vi "Return client handle.vi"(8 "error in (no error)":errorcluster, 9 "headers":T1[](array[typedef]), 10 "http-client":refnum<class "http-client.lvclass">, 11 "REST Client in":refnum<class "REST Client.lvclass">) -> (0 "error out":errorcluster, 3 "REST Client out":refnum<class "REST Client.lvclass">)   [LabVIEW 2020, in "REST Client.lvlib" / "REST Client.lvclass"]
uses:
  REST Client.lvclass
  http-client/http-client.lvclass
  HTTP Header.ctl
  <vilib>/NI/Advanced HTTP Client/Header--Combo Box.ctl
  REST Client.lvclass/REST Client.ctl
  <vilib>/NI/Advanced HTTP Client/Session.lvclass
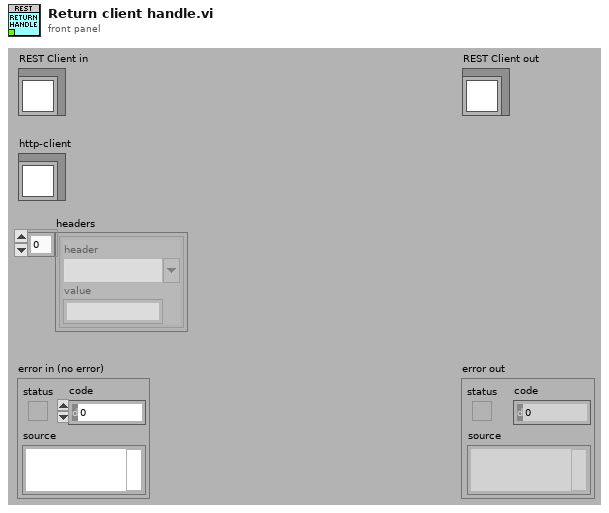
[diagram p1: front panel]
types:
  T1 = typedef "REST Client.lvlib/REST Client.lvclass/HTTP Header.ctl" = cluster{"header":T2, "value":string}
  T2 = typedef "lib_NI_Advanced HTTP Client.lvlib/Session.lvclass/Header--Combo Box.ctl" = string
  T3 = cluster{"http-client":refnum<class "http-client.lvclass">, "headers":T1[]}
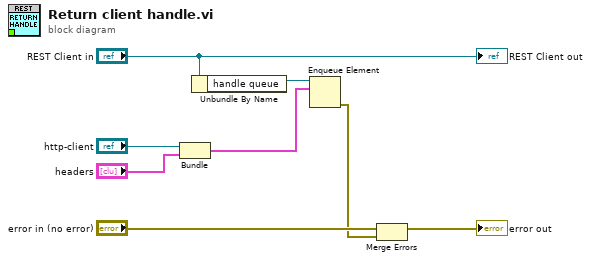
[diagram p0: block diagram]
diagram:
  n1 = Bundle("http-client"="http-client", "headers"="headers") -> (w5:T3)  [unwired: 1 in]
  n2 = Unbundle By Name("REST Client in") -> ("handle queue"=w6:refnum<queue>)
  n3 = Enqueue Element(queue=w6, element=w5) -> (error out=w3:errorcluster)  [unwired: 2 in, 2 out]
  n4 = Merge Errors("error in (no error)", w3) -> (→"error out":errorcluster)
  "REST Client out" <- "REST Client in"
